vi "Volt Detection.vi"(8 "error in":errorcluster, 11 "Voltage selection":T1) -> (0 "error out":errorcluster, 2 "Result":string, 3 "Result":bool)   [LabVIEW 2021]
uses:
  Voltage selection.ctl
  DUT/DUT_Cmd.ctl
  10054_Control Folder/Support/10054_states.ctl
panel:
  out "DUT Reading":bool
  out "number":dbl
  out "DMM Reading":bool
  out "Command Response":string
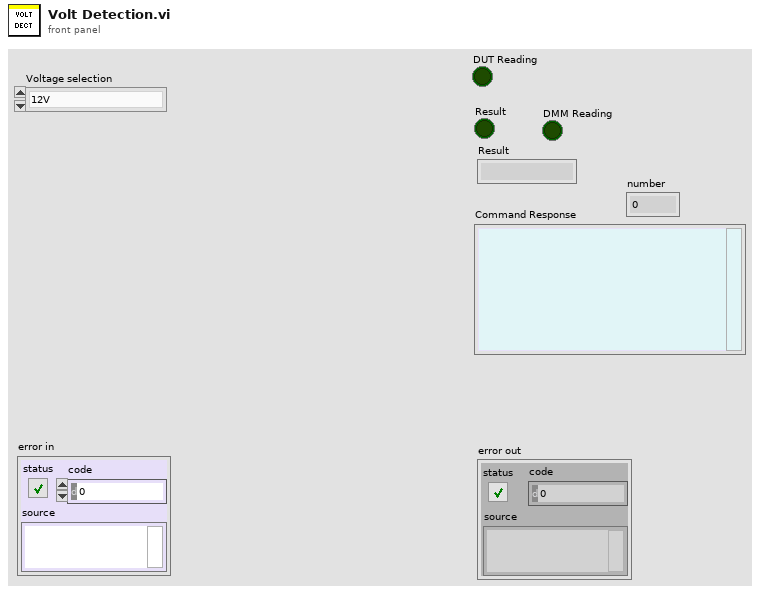
[diagram p1: front panel]
types:
  T1 = typedef "Voltage selection.ctl" = enum16{"12V", "5V", "3.3V"}
  T2 = typedef "DUT_Cmd.ctl" = enum16{"Unlock serial", "Stop console logs", "Release emergency at start", "Read firmware", "WiFi credentials", "WiFi connected", "WiFi SSID", "Board revision", "ADC_NTC_TEMP", "ADC_TYPE2_RCD_CURRENT", "PCBA serial write", "PCBA serial readback", "Start energy meter", "Energy meter Vac", "Energy meter Iac", "Energy meter PF", "Energy meter energy", "Provision", "Set gateway identity", "CP checklist", "Earth detect", "D+M sense unplugged", "D+M sense plugged", "Output relay weld", "Start diagnostics", "Relay 1 on", "Relay 2 on", "Emergency pressed", "Release emergency", "Emergency released", "Unlock serial for 5 A", "Board current (5 A)", "Unlock serial for 15 A", "Board current (15 A)", "Unlock serial for 0 A", "NFC tag", "Start diagnostics again", "Relay 2 off", "Relay 1 off", "End diagnostics", "Load current (5 A) [No USB station]", "Load current (15 A) [No USB station]", "Load current (0 A) [No USB station]", "NFC tag [No USB station]", "Battery Voltage", "FW Power reset", "Notification LED", "O/P Relay weld Detection", "Earth Detection", "12V ", "5V", "3.3V"}
  T3 = typedef "10054_states.ctl" = enum16{"Pilz-1", "Pilz-2", "AC CON - 2", "AC CON - 3", "AC CON - 4", "AC CON - 5", "Tower Lamp - Red", "Tower Lamp - Amber", "Tower Lamp - Green", "FAN 1 & 2", "FAN 3 & 4", "FAN 5 & 6", "Load - 1 10A", "Load - 2 10A", "Load - 3 5A", "Load - 4 5A", "Load - 5 2A", "TP49 - 12V", "TP20 - 5V", "TP148 - 3.3", "TP193 - GND", "J11.1 POS", "J11.2 NEG", "Noti LED POS", "Noti LED NEG", "Noti LED  5V", "D+M J14.1 - 3.3", "D+M J14.2 - GND", "NFC - 1", "NFC - 2"}
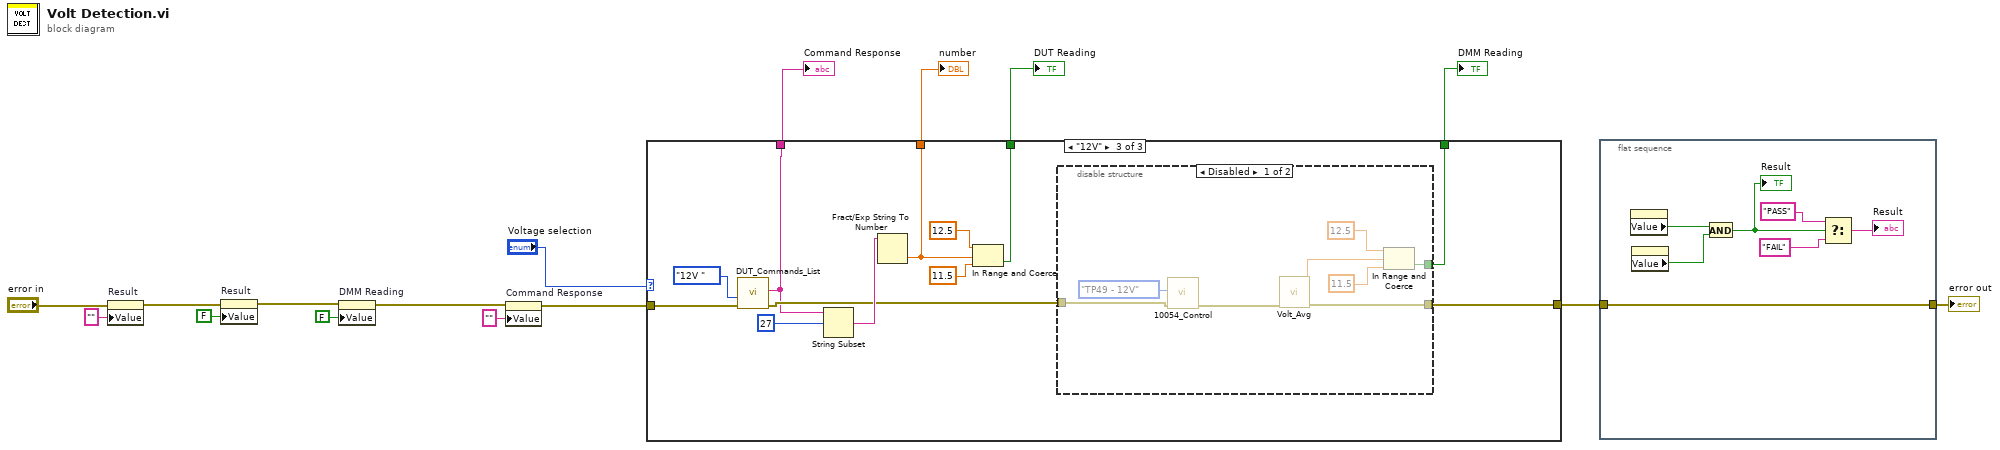
[diagram p0: block diagram]
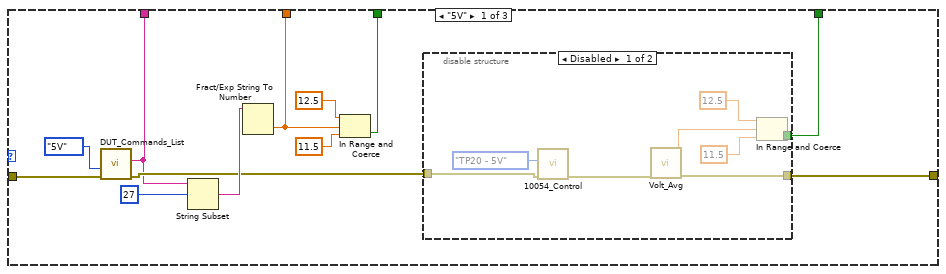
[diagram p2: hidden frame]
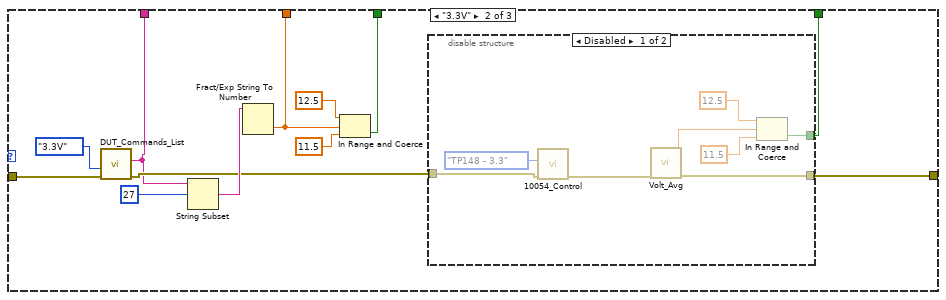
[diagram p4: hidden frame]
diagram:
  n1 = property on="Result" class="Str"(error in="error in", "Value"="" ("Result")) -> (error out=w9:errorcluster)  [unwired: 1 in, 1 out]
  n2 = property on="Result" class="Bool (strict)"(error in=w9, "Value"=FALSE ("DUT Reading")) -> (error out=w8:errorcluster)  [unwired: 1 in, 1 out]
  n3 = property on="DMM Reading" class="Bool (strict)"(error in=w8, "Value"=FALSE ("DMM Reading")) -> (error out=w7:errorcluster)  [unwired: 1 in, 1 out]
  n4 = property on="Command Response" class="Str"(error in=w7, "Value"="" ("Command Response")) -> (error out=w16:errorcluster)  [unwired: 1 in, 1 out]
  n5 = case shown="\"12V\"" "Voltage selection" {
    tunnel: w16 -> [w27 w47 w67]
    tunnel: [w24 w44 w64] -> w1
    tunnel: [w20 w40 w60] -> w14
    tunnel: [w19 w39 w59] -> w12
    tunnel: [w18 w38 w58] -> w3
    tunnel: [w17 w37 w57] -> w2
    frame "5V" {
      n6 = call "DUT_Commands_List.vi"("error in"=w27, "DUT Cmd"=DUT_Cmd."5V") -> ("error out"=w21:errorcluster, "Command Response"=w18:string)  [unwired: 7 in, 1 out]
      n7 = String Subset(string=w18, offset (0)=27) -> (substring=w25:string)  [unwired: 1 in]
      n8 = Fract/Exp String To Number(string=w25) -> (number=w17:dbl)  [unwired: 3 in, 1 out]
      n9 = In Range and Coerce(upper limit=12.5, x=w17, lower limit=11.5) -> (In Range?=w24:bool)  [unwired: 1 out]
      n10 = disable-structure shown="Disabled" {
        disable-tunnel: w21 -> [w36 _]
        disable-tunnel: [w30 _] -> w20
        disable-tunnel: [w29 _] -> w19
        frame Disabled {
          n11 = call "10054_Control.vi"("error in"=w36, "Pin"=10054_states."TP20 - 5V") -> ("error out"=w34:errorcluster)  [unwired: 5 in, 3 out]
          n12 = call "Volt_Avg.vi"("error in (no error)"=w34) -> ("error out"=w29:errorcluster, "x/Average"=w33:dbl)  [unwired: 9 in]
          n13 = In Range and Coerce(upper limit=12.5, x=w33, lower limit=11.5) -> (In Range?=w30:bool)  [unwired: 1 out]
        }
        frame Enabled {
        }
      }
    }
    frame "3.3V" {
      n14 = call "DUT_Commands_List.vi"("error in"=w47, "DUT Cmd"=DUT_Cmd."3.3V") -> ("error out"=w41:errorcluster, "Command Response"=w38:string)  [unwired: 7 in, 1 out]
      n15 = String Subset(string=w38, offset (0)=27) -> (substring=w45:string)  [unwired: 1 in]
      n16 = Fract/Exp String To Number(string=w45) -> (number=w37:dbl)  [unwired: 3 in, 1 out]
      n17 = In Range and Coerce(upper limit=12.5, x=w37, lower limit=11.5) -> (In Range?=w44:bool)  [unwired: 1 out]
      n18 = disable-structure shown="Disabled" {
        disable-tunnel: w41 -> [w56 _]
        disable-tunnel: [w50 _] -> w40
        disable-tunnel: [w49 _] -> w39
        frame Disabled {
          n19 = call "10054_Control.vi"("error in"=w56, "Pin"=10054_states."TP148 - 3.3") -> ("error out"=w54:errorcluster)  [unwired: 5 in, 3 out]
          n20 = call "Volt_Avg.vi"("error in (no error)"=w54) -> ("error out"=w49:errorcluster, "x/Average"=w53:dbl)  [unwired: 9 in]
          n21 = In Range and Coerce(upper limit=12.5, x=w53, lower limit=11.5) -> (In Range?=w50:bool)  [unwired: 1 out]
        }
        frame Enabled {
        }
      }
    }
    frame "12V" {
      n22 = call "DUT_Commands_List.vi"("error in"=w67, "DUT Cmd"=DUT_Cmd."12V ") -> ("error out"=w61:errorcluster, "Command Response"=w58:string)  [unwired: 7 in, 1 out]
      n23 = String Subset(string=w58, offset (0)=27) -> (substring=w65:string)  [unwired: 1 in]
      n24 = Fract/Exp String To Number(string=w65) -> (number=w57:dbl)  [unwired: 3 in, 1 out]
      n25 = In Range and Coerce(upper limit=12.5, x=w57, lower limit=11.5) -> (In Range?=w64:bool)  [unwired: 1 out]
      n26 = disable-structure shown="Disabled" {
        disable-tunnel: w61 -> [w76 _]
        disable-tunnel: [w70 _] -> w60
        disable-tunnel: [w69 _] -> w59
        frame Disabled {
          n27 = call "10054_Control.vi"("error in"=w76, "Pin"=10054_states."TP49 - 12V") -> ("error out"=w74:errorcluster)  [unwired: 5 in, 3 out]
          n28 = call "Volt_Avg.vi"("error in (no error)"=w74) -> ("error out"=w69:errorcluster, "x/Average"=w73:dbl)  [unwired: 9 in]
          n29 = In Range and Coerce(upper limit=12.5, x=w73, lower limit=11.5) -> (In Range?=w70:bool)  [unwired: 1 out]
        }
        frame Enabled {
        }
      }
    }
  }
  "DMM Reading" <- w14
  "Command Response" <- w3
  "number" <- w2
  "DUT Reading" <- w1
  n30 = flat-sequence {
    tunnel: w12 -> [w78]
    tunnel: [w78] -> w4
    frame #0 {
      n31 = property on="Result" class="Bool (strict)"() -> ("Value"=w80:bool)  [unwired: 2 in, 2 out]
      n32 = property on="DMM Reading" class="Bool (strict)"() -> ("Value"=w79:bool)  [unwired: 2 in, 2 out]
      n33 = And(x=w80, y=w79) -> (x .and. y?=w77:bool)
      "Result" <- w77
      n34 = Select(t="PASS", s=w77, f="FAIL") -> (s? t:f=→"Result":string)
    }
  }
  "error out" <- w4
